vi "Read TXT File.vi"(11 "File Path":path) -> (3 "数据系列":T1[](array[typedef]))   [LabVIEW 2020, in "Data Viewer.lvlib" / "Data Viewer.lvclass"]
uses:
  Data Viewer.lvclass
  Data Serie--cluster.ctl
  <vilib>/Utility/file.llb/Read Delimited Spreadsheet (string).vi
  Data Viewer.lvlib
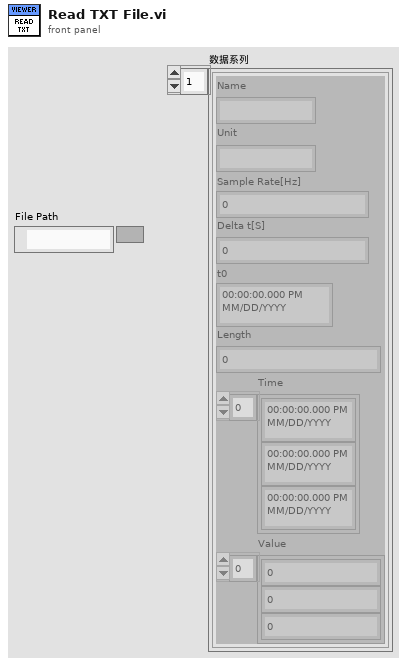
[diagram p1: front panel]
types:
  T1 = typedef "Data Viewer.lvlib/Data Serie--cluster.ctl" = cluster{"Name":string, "Unit":string, "Sample Rate[Hz]":dbl, "Delta t[S]":dbl, "t0":timestamp, "Length":i32, "Time":timestamp[], "Value":dbl[]}
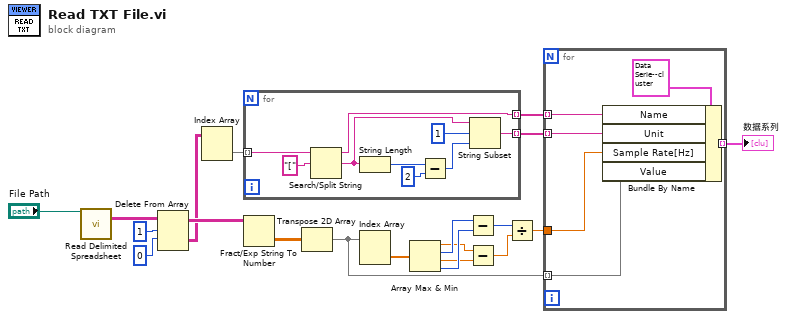
[diagram p0: block diagram]
diagram:
  n1 = call-poly <vilib>:"Read Delimited Spreadsheet.vi"("file path (dialog if empty)"="File Path") -> ("all rows"=w18:string[][])  [unwired: 9 in, 5 out]
  n2 = Delete From Array(array=w18, length=1 ("长度"), index (row)=0 ("索引 (行)")) -> (deleted portion=w4:string[][], array with subset deleted=w5:string[][])  [unwired: 1 in]
  n3 = Index Array(array=w4) -> (element=w6:string[])  [unwired: 2 in]
  n4 = for {
    tunnel: w6 -> [w29] mode=indexing
    tunnel: [w27] -> w8 mode=indexing
    tunnel: [w21] -> w9 mode=indexing
    n5 = Search/Split String(string=w29, search string/char (-)="[" ("搜索字符串/字符(-)")) -> (substring before match=w27:string, match + rest of string=w25:string)  [unwired: 1 in, 1 out]
    n6 = String Length(string=w25) -> (length=w23:i32)
    n7 = Subtract(x=w23, y=2) -> (x-y=w24:i32)
    n8 = String Subset(string=w25, offset (0)=1 ("偏移量(0)"), length (rest)=w24) -> (substring=w21:string)
  }
  n9 = Fract/Exp String To Number(string=w5) -> (number=w7:dbl[][])  [unwired: 3 in, 1 out]
  n10 = Transpose 2D Array(2D array=w7) -> (transposed array=w10:dbl[][])
  n11 = Index Array(array=w10) -> (element=w11:dbl[])  [unwired: 2 in]
  n12 = Array Max & Min(array=w11) -> (max value=w12:dbl, max index (indices)=w14:i32, min value=w13:dbl, min index (indices)=w15:i32)
  n13 = Subtract(x=w14, y=w15) -> (x-y=w20:i32)
  n14 = Subtract(x=w12, y=w13) -> (x-y=w19:dbl)
  n15 = Divide(x=w20, y=w19) -> (x/y=w16:dbl)
  n16 = for {
    tunnel: w8 -> [w35] mode=indexing
    tunnel: w9 -> [w34] mode=indexing
    tunnel: w10 -> [w33] mode=indexing
    tunnel: w16 -> [w32]
    tunnel: [w31] -> w17 mode=indexing
    n17 = Bundle By Name(cluster=T1 {"Name"="", "Unit"="", "Sample Rate[Hz]"=0.0, "Delta t[S]"=0.0, "t0"=timestamp(0 s since 1904-01-01), "Length"=0, "Time"=[], "Value"=[]} ("Data Serie"), "Name"=w35, "Unit"=w34, "Sample Rate[Hz]"=w32, "Value"=w33) -> (w31:T1)
  }
  "数据系列" <- w17
